vi "test Loopback.vi"(8 "error in (no error)":errorcluster, 11 "TestCase in":refnum<class "SLSC EDS System Tests.lvclass">) -> (0 "error out":errorcluster, 3 "TestCase out":refnum<class "SLSC EDS System Tests.lvclass">)   [LabVIEW 2020, in "SLSC EDS System Tests.lvclass"]
uses:
  SLSC EDS System Tests.lvclass
  C:/Program Files (x86)/National Instruments/LabVIEW 2020/vi.lib/NI/VeriStand Custom Device Testing Tools/VeriStandTestCase/VeriStandTestCase.lvclass
  C:/Program Files (x86)/National Instruments/LabVIEW 2020/vi.lib/addons/_JKI Toolkits/VI Tester/TestCase.llb/TestCase.lvclass
  Loopback/Loopback.lvclass
  <vilib>/addons/_JKI Toolkits/VI Tester/TestCase.llb/TestCase.lvclass
  <vilib>/NI/VeriStand Custom Device Testing Tools/VeriStandTestCase/VeriStandTestCase.lvclass
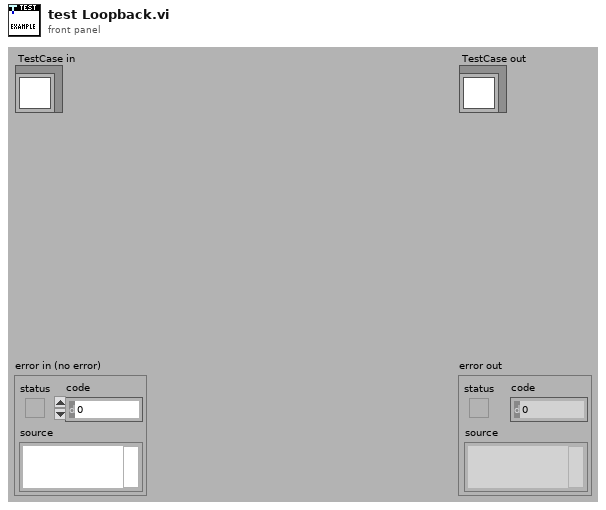
[diagram p1: front panel]
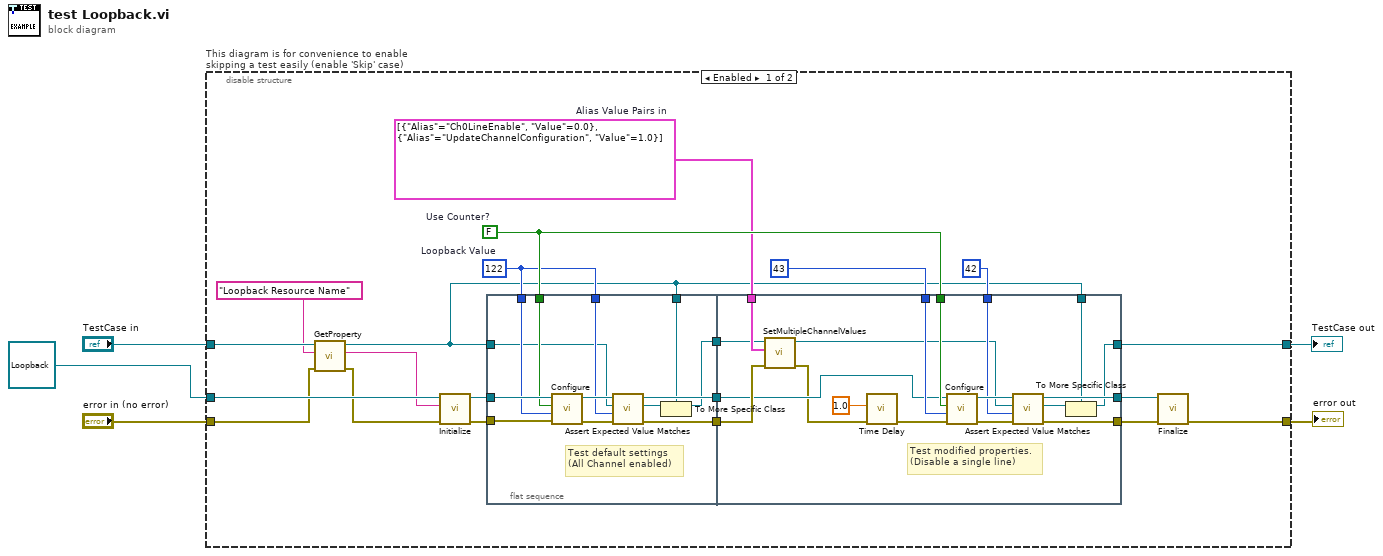
[diagram p0: block diagram]
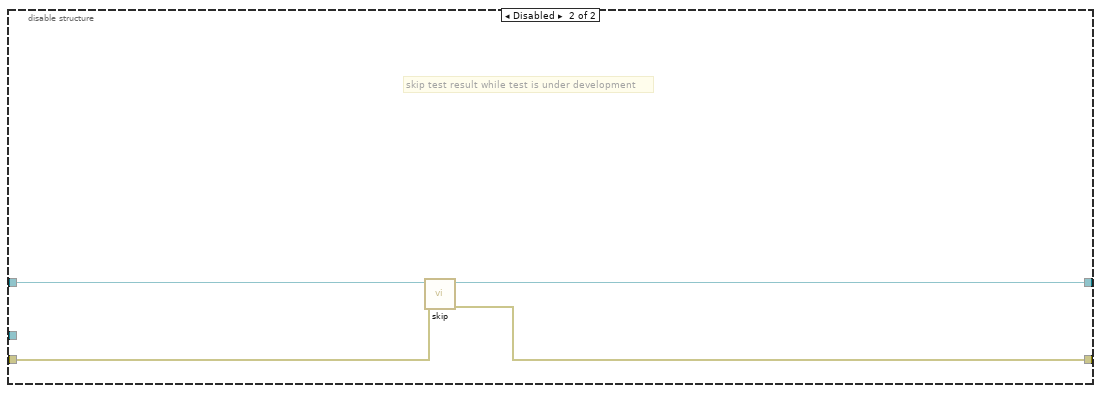
[diagram p2: hidden frame]
diagram:
  n1 = disable-structure "This diagram is for convenience to enable skipping a test easily (enable 'Skip' case)" shown="Enabled" {
    disable-tunnel: "TestCase in" -> [w11 w61]
    disable-tunnel: [w13 w59] -> w1
    disable-tunnel: [w15 w60] -> w4
    disable-tunnel: "error in (no error)" -> [w9 w58]
    disable-tunnel: refnum<class "Loopback.lvclass"> refnum ("Loopback.lvclass") -> [w21 _]
    frame Enabled {
      w25 = cluster{"Alias":string, "Value":dbl}[] [{"Alias"="Ch0LineEnable", "Value"=0.0}, {"Alias"="UpdateChannelConfiguration", "Value"=1.0}]  # Alias Value Pairs in
      w22 = u8 122  # Loopback Value
      w26 = FALSE  # Use Counter?
      n2 = call <vilib>:"GetProperty.vi"("error in (no error)"=w9, "key"="Loopback Resource Name", "VeriStandTestCase in"=w11) -> ("error out"=w8:errorcluster, "value"=w7:string, "VeriStandTestCase out"=w10:refnum<class "SLSC EDS System Tests.lvclass">)  [unwired: 6 in]
      n3 = call-dynamic "Initialize.vi"("error in (no error)"=w8, "Resource Name in"=w7, "Loopback in"=w21) -> ("error out"=w20:errorcluster, "Loopback out"=w19:refnum<class "Loopback.lvclass">)  [unwired: 7 in]
      n4 = flat-sequence {
        tunnel: w10 -> [w30]
        tunnel: w20 -> [w38]
        tunnel: w22 -> [w37]
        tunnel: w26 -> [w36]
        tunnel: w22 -> [w31]
        tunnel: w19 -> [w39]
        tunnel: [w33] -> w18
        tunnel: [w32] -> w17
        tunnel: [w28] -> w12
        tunnel: w10 -> [w27]
        tunnel: w26 -> [w55]
        tunnel: w25 -> [w50]
        tunnel: u8 43 ("Value") -> [w56]
        tunnel: u8 42 ("Expected Value") -> [w52]
        tunnel: w18 -> [w49]
        tunnel: w17 -> [w43]
        tunnel: [w54] -> w16
        tunnel: [w51] -> w14
        tunnel: [w46] -> w13
        tunnel: w12 -> [w47]
        tunnel: w10 -> [w44]
        frame #0 {
          # "Test default settings\n(All Channel enabled)"
          n5 = call-dynamic "Configure.vi"("error in (no error)"=w38, "Value in"=w37, "Use Counter?"=w36, "Loopback in"=w39) -> ("error out"=w34:errorcluster, "Loopback out"=w35:refnum<class "Loopback.lvclass">)  [unwired: 6 in]
          n6 = call-dynamic "Assert Expected Value Matches.vi"("error in (no error)"=w34, "Expected Value"=w31, "TestCase in"=w30, "Loopback in"=w35) -> ("error out"=w33:errorcluster, "TestCase out"=w29:refnum<class "TestCase.lvclass">, "Loopback out"=w32:refnum<class "Loopback.lvclass">)  [unwired: 5 in]
          n7 = To More Specific Class(target class=w27, reference=w29) -> (specific class reference=w28:refnum<class "SLSC EDS System Tests.lvclass">)  [unwired: 1 in, 1 out]
        }
        frame #1 {
          # "Test modified properties.\n(Disable a single line)"
          n8 = call-dynamic "SetMultipleChannelValues.vi"("error in (no error)"=w49, "Channel Key Value Pairs in"=w50, "VeriStandTestCase in"=w47) -> ("error out"=w41:errorcluster, "VeriStandTestCase out"=w48:refnum<class "SLSC EDS System Tests.lvclass">)  [unwired: 7 in]
          n9 = call "Time Delay"("error in (no error)"=w41, "Delay Time (s)"=1.0) -> ("error out"=w42:errorcluster)  [unwired: 9 in]
          n10 = call-dynamic "Configure.vi"("error in (no error)"=w42, "Value in"=w56, "Use Counter?"=w55, "Loopback in"=w43) -> ("error out"=w57:errorcluster, "Loopback out"=w53:refnum<class "Loopback.lvclass">)  [unwired: 6 in]
          n11 = call-dynamic "Assert Expected Value Matches.vi"("error in (no error)"=w57, "Expected Value"=w52, "TestCase in"=w48, "Loopback in"=w53) -> ("error out"=w54:errorcluster, "TestCase out"=w45:refnum<class "TestCase.lvclass">, "Loopback out"=w51:refnum<class "Loopback.lvclass">)  [unwired: 5 in]
          n12 = To More Specific Class(target class=w44, reference=w45) -> (specific class reference=w46:refnum<class "SLSC EDS System Tests.lvclass">)  [unwired: 1 in, 1 out]
        }
      }
      n13 = call-dynamic "Finalize.vi"("error in (no error)"=w16, "Loopback in"=w14) -> ("error out"=w15:errorcluster)  [unwired: 8 in, 1 out]
    }
    frame Disabled {
      # "skip test result while test is under development"
      n14 = call <vilib>:"skip.vi"("error in (no error)"=w58, "TestCase in"=w61) -> ("error out"=w60:errorcluster, "TestCase out"=w59:refnum<class "SLSC EDS System Tests.lvclass">)  [unwired: 8 in]
    }
  }
  "error out" <- w4
  "TestCase out" <- w1
